vi "RichToFlatcif_can_writer_cansub_CanMessage.vi"(5 "OutputClusterType":T1, 11 "InputCluster":T2) -> (3 "OutputCluster":T1)   [LabVIEW 2021, in "CanWriterCansub_client.lvlib"]
uses:
  CanWriterCansub_client.lvlib
  cif_can_writer_cansub_CanMessage.ctl
  cif_can_writer_cansub_CanMessage_Flat.ctl
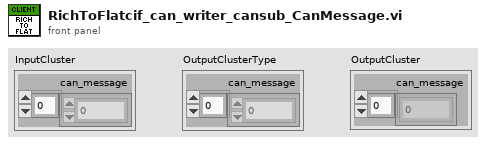
[diagram p1: front panel]
types:
  T1 = typedef "CanWriterCansub_client.lvlib/cif_can_writer_cansub_CanMessage_Flat.ctl" = cluster{"can_message":u8[]}
  T2 = typedef "CanWriterCansub_client.lvlib/cif_can_writer_cansub_CanMessage.ctl" = cluster{"can_message":u8[]}
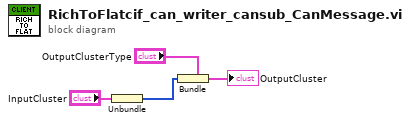
[diagram p0: block diagram]
diagram:
  n1 = Unbundle "Unbundle"("InputCluster") -> ("can_message"=w1:u8[])
  n2 = Bundle "Bundle"(cluster="OutputClusterType", "can_message"=w1) -> (→"OutputCluster":T1)
